vi "Event handler-Ref laser power change.vi"(10 "Ref Laser Power":u8) -> ()   [LabVIEW 2020]
uses:
  Peripherals Control/Pockels/Globals/gl_Pockels control globals.vi
  Global Variables/gl_UI Ctrl Refs.vi
  Global Variables/General Globals.vi
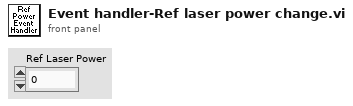
[diagram p1: front panel]
types:
  T1 = typedef "UI ctrl refs cluster.ctl" = cluster{"Top level VI path":path, "Top level VI ref":refnum<vi>, "User menu ref":refnum<k9>, "Sub Panel control":refnum<vi>, "Imaging Param Tab":refnum<vi>, "Occurrence-Start drivers":refnum<k4>, "Occurrence-Speed logging initialised":refnum<k4>, "Occurrence-XYZ stage initialised":refnum<k4>, "Exit button":refnum<vi>, "Status ind":refnum<vi>, "Set as origin":refnum<vi>, "Speed Logging":refnum<vi>, "Time Lapse":refnum<vi>, "Live Imaging":refnum<vi>, "AOL Z Stack":refnum<vi>, "Motor Z Stack":refnum<vi>, "Funct Acq button":refnum<vi>, "Hard Shutter":refnum<vi>, "Virtual Shutter":refnum<vi>, "Laser Power":refnum<vi>, "AOL Mode":refnum<vi>, "Frame Size":refnum<vi>, "Field of View":refnum<vi>, "Dwell Time":refnum<vi>, "Zoom":refnum<vi>, "AOL Z":refnum<vi>, "Objective":refnum<vi>, "Axis":refnum<vi>, "Paths & Names":refnum<vi>, "Experiment folder path (ind.)":refnum<vi>, "Last State (Ind.)":refnum<vi>, "Averages":refnum<vi>, "Angle (degrees)":refnum<vi>, "X centre":refnum<vi>, "Y centre":refnum<vi>, "Plane Mode":refnum<vi>, "# Planes":refnum<vi>, "Z Start":refnum<vi>, "Z Stop":refnum<vi>, "Z Step":refnum<vi>, "PMT 1":refnum<vi>, "PMT 2":refnum<vi>, "Stage XYZ Position":refnum<vi>, "Pockels@Z Start":refnum<vi>, "Pockels@Z Stop":refnum<vi>, "Obtain Z Start":refnum<vi>, "Obtain Z Stop":refnum<vi>, "Live stim.trig.period":refnum<vi>, "Live stim.trig.enable":refnum<vi>, "Movement Correction":refnum<vi>, "Load Reference Image":refnum<vi>, "XY Stage Move":refnum<vi>, "MovCor Cluster":refnum<vi>, "RefDAQParam":refnum<vi>, "Funct. Acq. Pockels Modulation":refnum<vi>, "Ref Laser Power":refnum<vi>, "Enable Video Recording":refnum<vi>, "Video Record-Live Imaging":refnum<vi>, "Video Record-Funct acq":refnum<vi>, "Reference Source":refnum<vi>, "AOL Z-stack Chirps Ready (ind)":refnum<vi>, "Target time between mov.cor. ref triggers (ms)":refnum<vi>, "Funct. Acq. Ref frame save":refnum<vi>, "Tracking button":refnum<vi>, "Show ref plots window":refnum<vi>, "Center freq ind (nm)":refnum<vi>, "Pickup mode (ind)":refnum<vi>, "Logging queue (ind)":refnum<vi>, "Back aperture power (ind.)":refnum<vi>, "Power after objective (ind.)":refnum<vi>, "Switch user":refnum<vi>, "Ls1 Conn. Status":refnum<vi>, "Ls1Tuning Status":refnum<vi>, "Ls1 Faults":refnum<vi>, "Ls1 Connection":refnum<vi>, "Ls1 Mode":refnum<vi>, "Ls1 POWER [mW]":refnum<vi>, "Ls1Shutter":refnum<vi>, "Ls1 Wavelength":refnum<vi>, "Ls1 Note":refnum<vi>, "Ls1 Confirm Wav":refnum<vi>, "Ls1 PreChrp Prism1":refnum<vi>, "Ls1 PreChrp Prism2":refnum<vi>, "Ls1 wav top Ind":refnum<vi>, "Ls1 power top Ind":refnum<vi>, "Ls1 Pump peak Hold":refnum<vi>, "Ls1 Status Ind":refnum<vi>, "Ls1 wav cancel":refnum<vi>, "Experiment Type":refnum<vi>, "Biology Information":refnum<vi>, "Camera recording status":refnum<vi>}
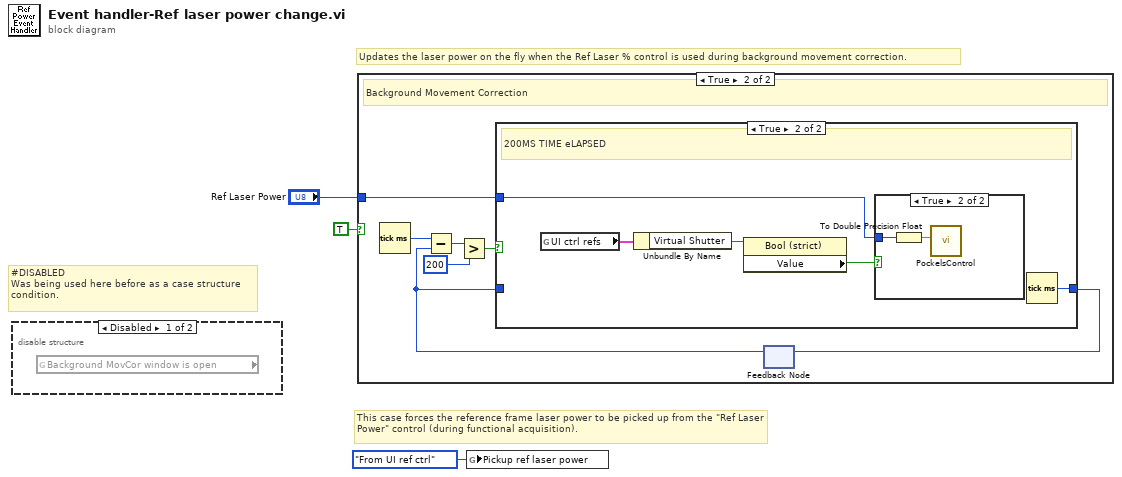
[diagram p0: block diagram]
diagram:
  # "#DISABLED\nWas being used here before as a case structure\ncondition."
  # "This case forces the reference frame laser power to be picked up from the \"Ref Laser Power\" control (during functional acquisition)."
  # "Updates the laser power on the fly when the Ref Laser % control is used during background movement correction."
  n1 = disable-structure shown="Disabled" {
    frame Disabled {
      n2 = global read "General Globals.vi" "Background MovCor window is open"() -> ()  [unwired: 1 out]
    }
    frame Enabled {
    }
  }
  n3 = case shown="True" TRUE {
    tunnel: "Ref Laser Power" -> [_ w10]
    frame False {
    }
    frame True {
      # "Background Movement Correction"
      n4 = Tick Count (ms)() -> (millisecond timer value=w5:u32)
      n5 = feedback #1() -> (w9:u32)  [unwired: 1 in]
      n6 = Subtract(x=w5, y=w9) -> (x-y=w6:u32)
      n7 = Greater?(x=w6, y=u32 200) -> (0:w8:bool)
      n8 = case shown="True" w8 {
        tunnel: w10 -> [_ w13]
        tunnel: [w11 w16] -> w4
        tunnel: w9 -> [w11 _]
        frame False {
        }
        frame True {
          # "200MS TIME eLAPSED"
          n9 = global read "gl_UI Ctrl Refs.vi" "UI ctrl refs"() -> (w12:T1)
          n10 = Unbundle By Name(w12) -> ("Virtual Shutter"=w15:refnum<vi>)
          n11 = property class="Bool (strict)"(reference=w15) -> ("Value"=w14:bool)  [unwired: 1 in, 2 out]
          n12 = case shown="True" w14 {
            tunnel: w13 -> [_ w18]
            frame False {
            }
            frame True {
              n13 = To Double Precision Float(number=w18) -> (double precision float=w17:dbl)
              n14 = call "PockelsControl.vi"("Laser Power (%)"=w17) -> ()  [unwired: 10 in, 1 out]
            }
          }
          n15 = Tick Count (ms)() -> (millisecond timer value=w16:u32)
        }
      }
      n16 = feedback-in #1(w4) -> ()
    }
  }
  n17 = global write "gl_Pockels control globals.vi" "Pickup ref laser power"(enum16{"From source image", "From UI ref ctrl"}."From UI ref ctrl" ("Pickup ref laser power")) -> ()
